vi "Main.vi"() -> ()   [LabVIEW 2021]
uses:
  Type defs/Parameters.ctl
  Type defs/Error FGV States.ctl
panel:
  out "image_num":i32
  in  "Stop":bool
  in  "Scanning options":enum32{"Item 0", "Item 1"}(radio)
  in  "Save to file":bool
  in  "Scanning":bool
  out "Errors":string
  in  "Saving data":T1
  out "Image Parameters":cluster{"Mean":dbl, "Offset":dbl}
  out "Intensity Graph":dbl[][](graph)
  in  "Parameters":T2={"Time"=0.0, "Pixels X"=1, "Pixels Y"=1, "Max galvo"=0.0, "Min galvo"=0.0} {"Pixels Y" min=1; "Pixels X" min=1 step=1; "Time" min=1.0}
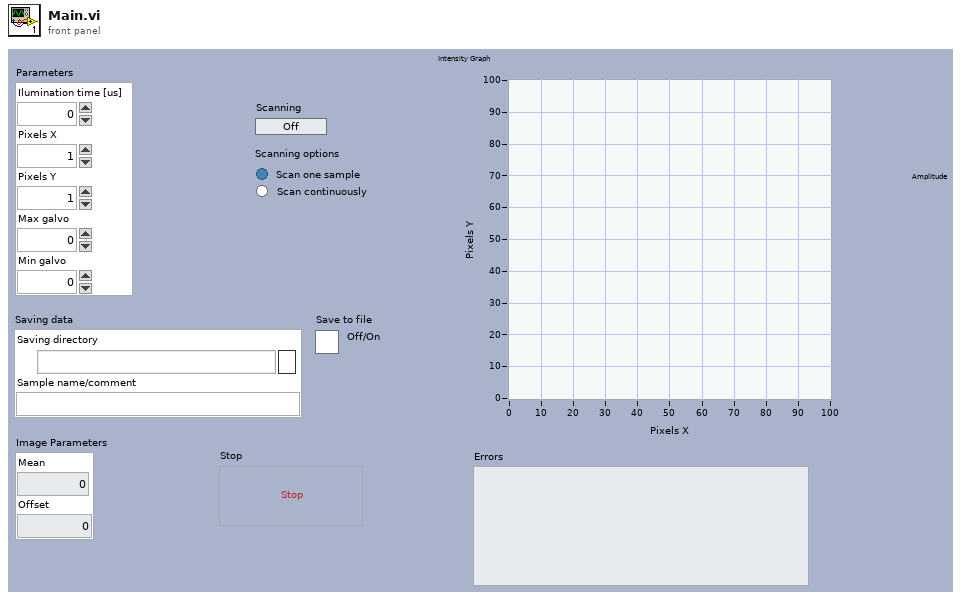
[diagram p1: front panel]
types:
  T1 = cluster{"Saving directory":path, "Sample name/comment":string}
  T2 = typedef "Parameters.ctl" = cluster{"Time":dbl, "Pixels X":i32, "Pixels Y":i32, "Max galvo":dbl, "Min galvo":dbl}
  T3 = typedef "Notifiers.ctl" = cluster{"DAQ notifier":refnum<notifier>, "Data notifier":refnum<notifier>}
  T4 = typedef "Queues.ctl" = cluster{"MHL":refnum<queue>, "DAQ":refnum<queue>, "Data":refnum<queue>, "Error":refnum<queue>}
  T5 = typedef "Error FGV States.ctl" = enum16{"Save", "Clear", "Add", "Read"}
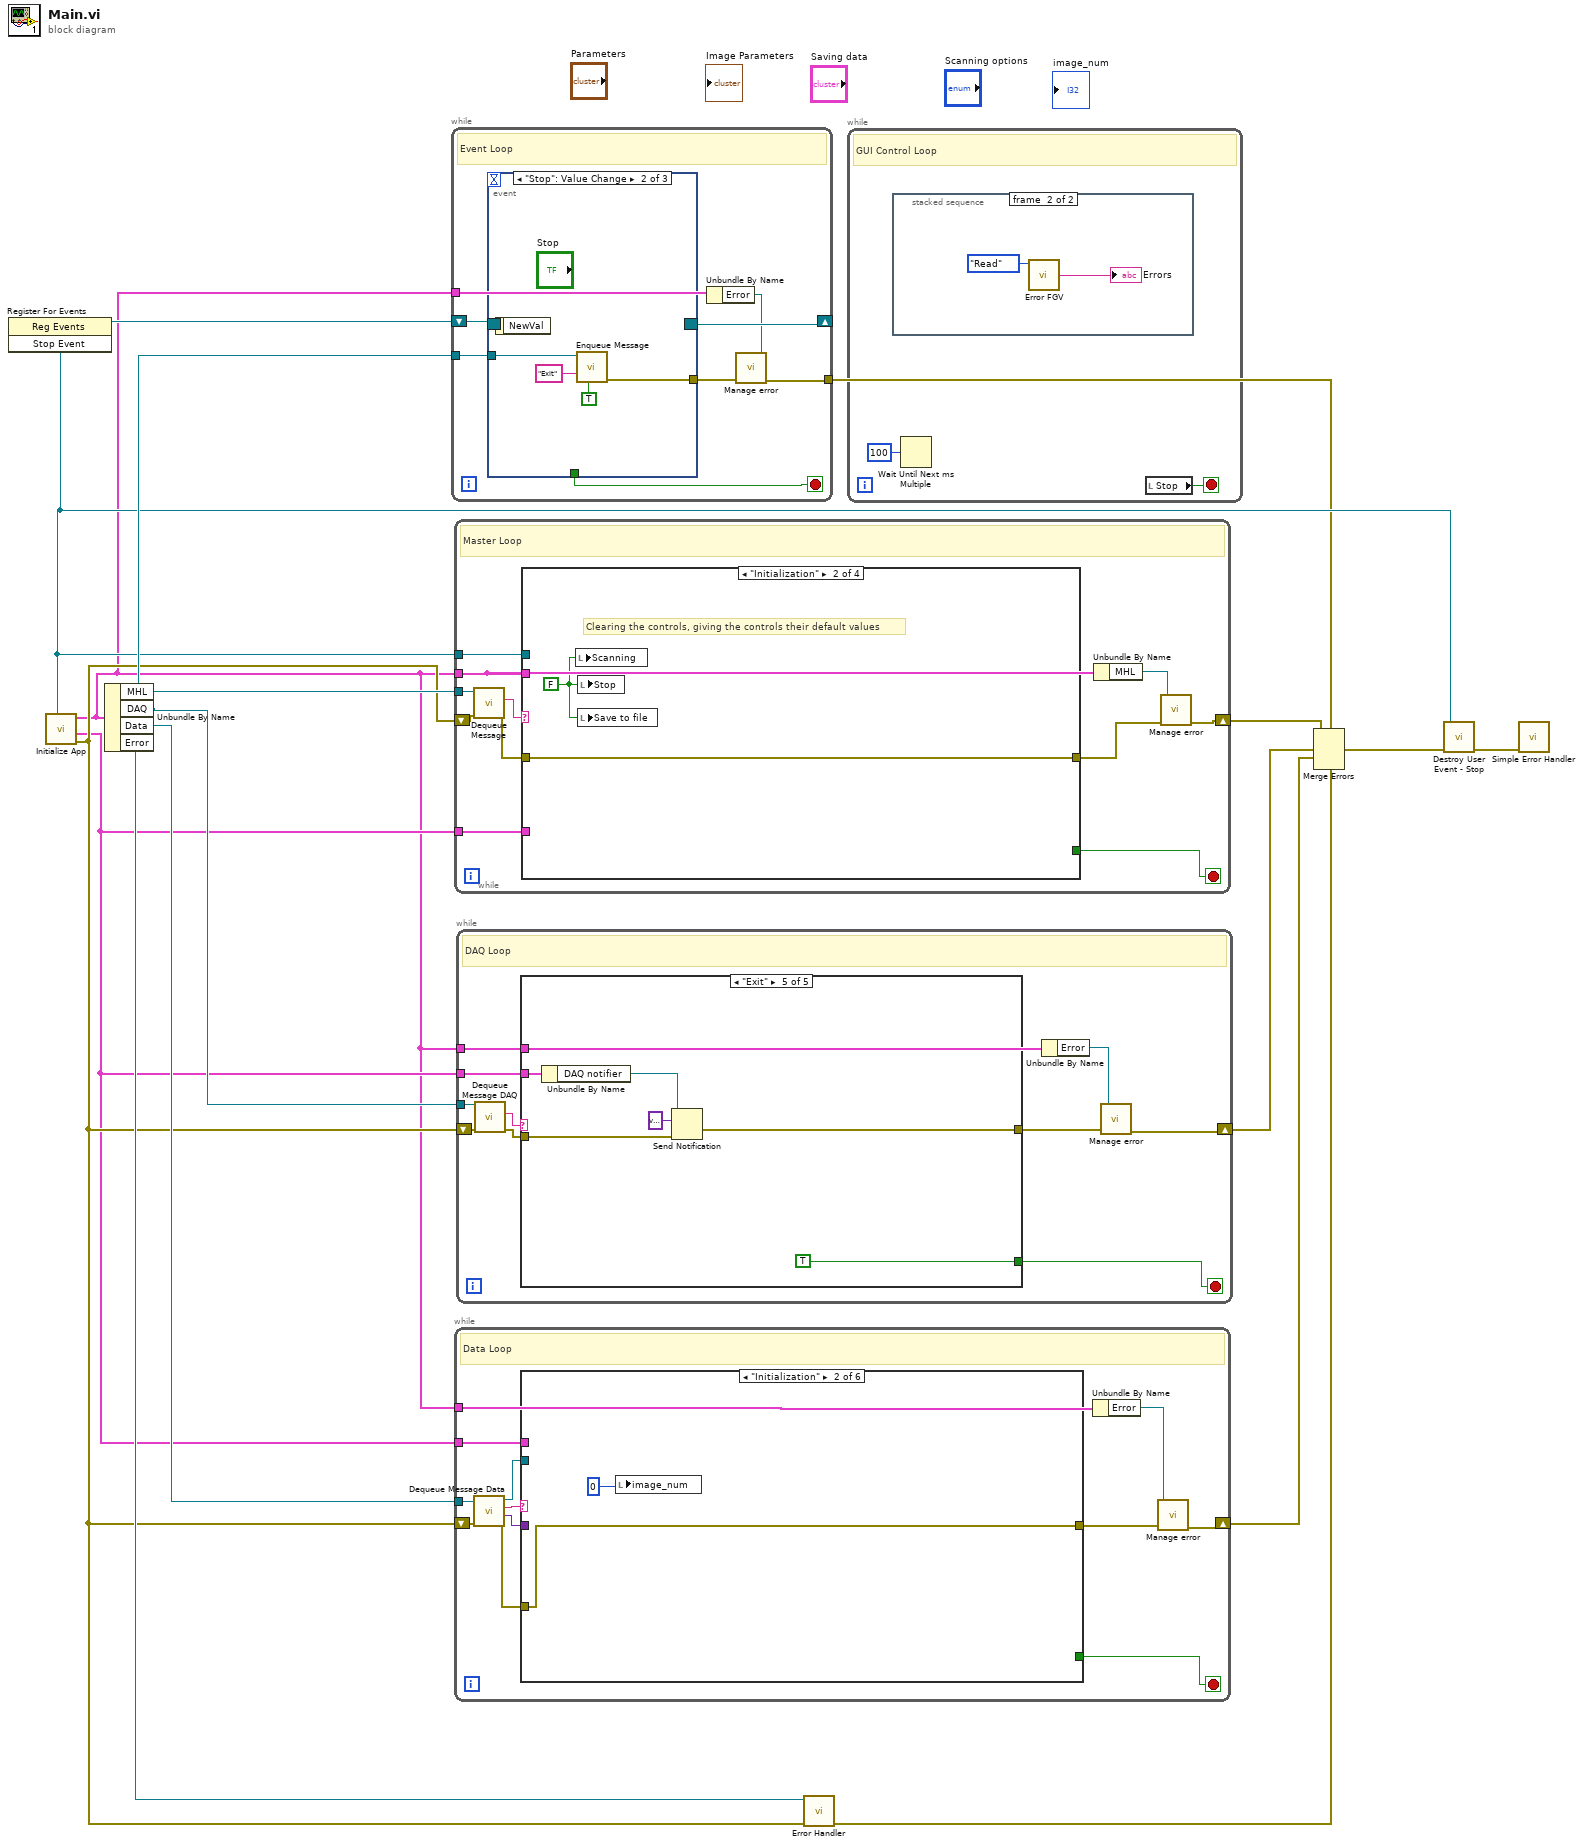
[diagram p0: block diagram]
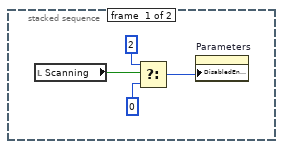
[diagram p2: hidden frame]
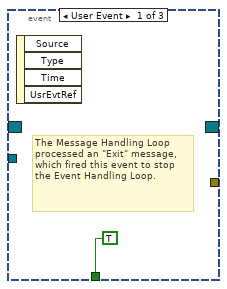
[diagram p3: hidden frame]
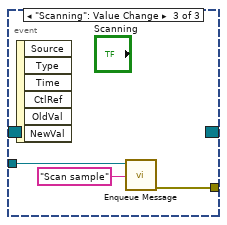
[diagram p4: hidden frame]
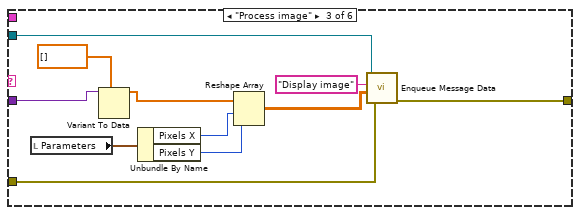
[diagram p6: hidden frame]
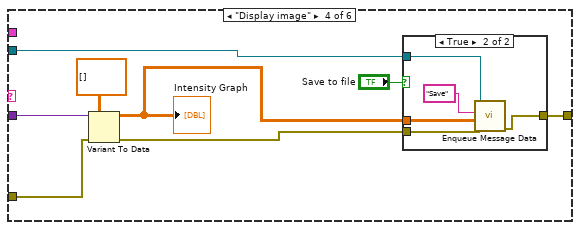
[diagram p7: hidden frame]
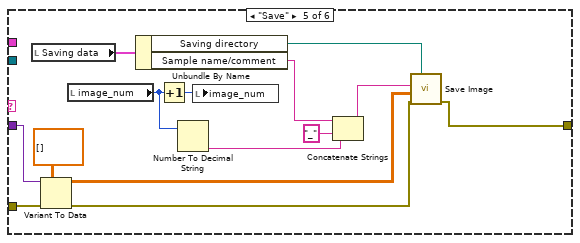
[diagram p9: hidden frame]
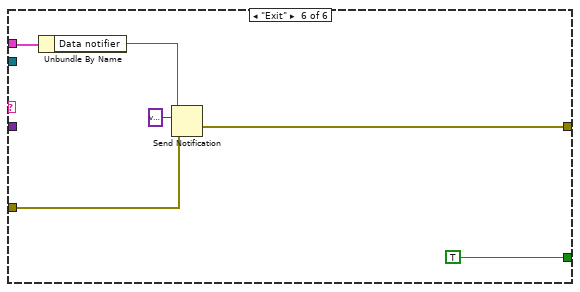
[diagram p10: hidden frame]
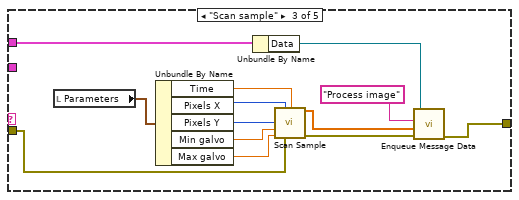
[diagram p13: hidden frame]
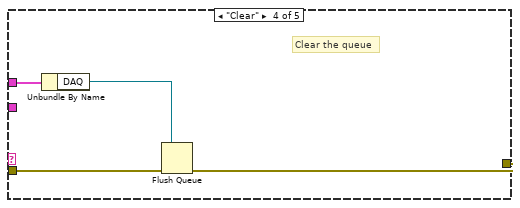
[diagram p14: hidden frame]
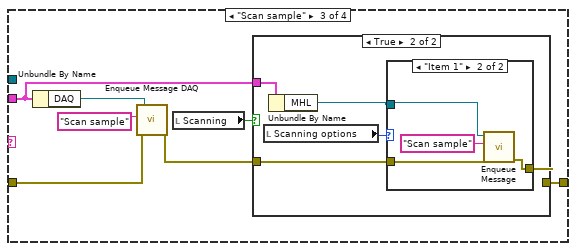
[diagram p16: hidden frame]
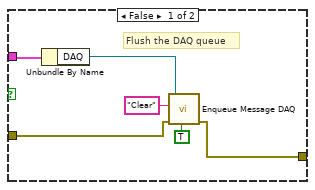
[diagram p17: hidden frame]
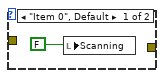
[diagram p18: hidden frame]
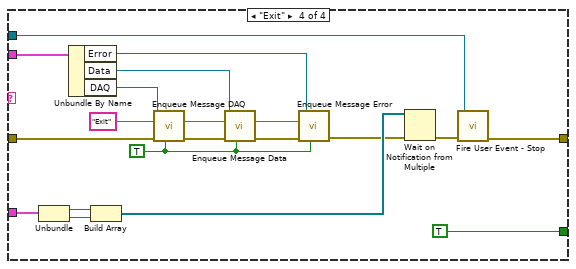
[diagram p19: hidden frame]
diagram:
  n1 = call "Initialize App.vi"() -> ("error out"=w10:errorcluster, "notifier cluster"=w2:T3, "Stop Event"=w11:refnum<user-event>, "queue cluster"=w1:T4)  [unwired: 8 in]
  n2 = register-events(w11) -> (reference out=w12:refnum<event-registration>)  [unwired: 2 in, 1 out]
  n3 = Unbundle By Name(w1) -> ("MHL"=w16:refnum<queue>, "DAQ"=w15:refnum<queue>, "Data"=w14:refnum<queue>, "Error"=w13:refnum<queue>)
  n4 = while {
    tunnel: w16 -> [w24]
    shift-right: [w22] -> _
    shift-left: w12 -> [w23]
    tunnel: [w19] -> w9
    tunnel: w1 -> [w18]
    stop <- w21 stop-if-true
    # "Event Loop"
    n5 = event shown="[1] \"Stop\": Value Change" {
      selector: w23 -> [_ _ _]
      dyn-events: [_ _ _] -> w22
      timeout: _ -> [_ _ _]
      tunnel: w24 -> [_ w29 w32]
      tunnel: [_ w28 w30] -> w20
      tunnel: [TRUE _ _] -> w21
      event User Event {
        # "The Message Handling Loop processed an \"Exit\" message, which fired this event to stop the Event Handling Loop."
        n6 = event-data() -> ()  [unwired: 1 in, 4 out]
      }
      event "Stop": Value Change {
        n7 = event-data() -> ()  [unwired: 1 in, 1 out]
        n8 = call "Enqueue Message.vi"("Priority message (F)"=TRUE, "Message"="Exit", "queue in"=w29) -> ("error out"=w28:errorcluster)  [unwired: 7 in, 1 out]
      }
      event "Scanning": Value Change {
        n9 = event-data() -> ()  [unwired: 1 in, 6 out]
        n10 = call "Enqueue Message.vi"("Message"="Scan sample", "queue in"=w32) -> ("error out"=w30:errorcluster)  [unwired: 8 in, 1 out]
      }
    }
    n11 = Unbundle By Name(w18) -> ("Error"=w17:refnum<queue>)
    n12 = call "Manage error.vi"("error in"=w20, "Error"=w17) -> ("error out"=w19:errorcluster)  [unwired: 9 in]
  }
  n13 = while {
    tunnel: w16 -> [w43]
    tunnel: w11 -> [w41]
    tunnel: w1 -> [w34]
    shift-right: [w35] -> w8
    shift-left: w10 -> [w38]
    tunnel: w2 -> [w37]
    stop <- w40 stop-if-true
    # "Master Loop"
    n14 = call "Dequeue Message.vi"("error in (no error)"=w38, "Message Queue"=w43) -> ("error out"=w39:errorcluster, "Message"=w42:string)  [unwired: 6 in, 2 out]
    n15 = case shown="\"Initialization\"" w42 {
      tunnel: w41 -> [_ _ _ w86]
      tunnel: [_ _ _ TRUE] -> w40
      tunnel: w34 -> [_ _ w49 w85]
      tunnel: w39 -> [w44 w46 w52 w79]
      tunnel: [w44 w46 w50 w76] -> w36
      tunnel: w37 -> [_ _ _ w75]
      frame Default {
      }
      frame "Initialization" {
        w45 = FALSE
        # "Clearing the controls, giving the controls their default values"
        n16 = local write "Scanning"(w45) -> ()
        n17 = local write "Stop"(w45) -> ()
        n18 = local write "Save to file"(w45) -> ()
      }
      frame "Scan sample" {
        n19 = Unbundle By Name(w49) -> ("DAQ"=w53:refnum<queue>)
        n20 = call "Enqueue Message DAQ.vi"("error in (no error)"=w52, "Message"="Scan sample", "queue in"=w53) -> ("error out"=w48:errorcluster)  [unwired: 7 in, 1 out]
        n21 = local read "Scanning"() -> (w47:bool)
        n22 = case shown="True" w47 {
          tunnel: [w56 w63] -> w50
          tunnel: w49 -> [w59 w62]
          tunnel: w48 -> [w57 w60]
          frame False {
            # "Flush the DAQ queue"
            n23 = Unbundle By Name(w59) -> ("DAQ"=w58:refnum<queue>)
            n24 = call "Enqueue Message DAQ.vi"("Priority message (F)"=TRUE, "error in (no error)"=w57, "Message"="Clear", "queue in"=w58) -> ("error out"=w56:errorcluster)  [unwired: 6 in, 1 out]
          }
          frame True {
            n25 = local read "Scanning options"() -> (w64:enum32{"Item 0", "Item 1"})
            n26 = Unbundle By Name(w62) -> ("MHL"=w61:refnum<queue>)
            n27 = case shown="\"Item 1\"" w64 {
              tunnel: [_ w69] -> w63
              tunnel: w61 -> [_ w68]
              tunnel: w60 -> [_ w66]
              frame "Item 0", Default {
                n28 = local write "Scanning"(FALSE) -> ()
              }
              frame "Item 1" {
                n29 = call "Enqueue Message.vi"("error in (no error)"=w66, "Message"="Scan sample", "queue in"=w68) -> ("error out"=w69:errorcluster)  [unwired: 7 in, 1 out]
              }
            }
          }
        }
      }
      frame "Exit" {
        w80 = TRUE ("Priority message (F)")
        w81 = "Exit"
        n30 = Unbundle(w75) -> ("DAQ notifier"=w74:refnum<notifier>, "Data notifier"=w73:refnum<notifier>)
        n31 = Unbundle By Name(w85) -> ("Error"=w82:refnum<queue>, "Data"=w83:refnum<queue>, "DAQ"=w84:refnum<queue>)
        n32 = Build Array(w74, w73) -> (w72:refnum<notifier>[])
        n33 = call "Enqueue Message DAQ.vi"("Priority message (F)"=w80, "error in (no error)"=w79, "Message"=w81, "queue in"=w84) -> ("error out"=w78:errorcluster)  [unwired: 6 in, 1 out]
        n34 = call "Enqueue Message Data.vi"("Priority message (F)"=w80, "error in (no error)"=w78, "Message"=w81, "queue in"=w83) -> ("error out"=w77:errorcluster)  [unwired: 6 in, 1 out]
        n35 = call "Enqueue Message Error.vi"("Priority message (F)"=w80, "error in (no error)"=w77, "Message"=w81, "queue in"=w82) -> ("error out"=w71:errorcluster)  [unwired: 6 in, 1 out]
        n36 = Wait on Notification from Multiple(0:w72, 3:w71) -> (11:w70:errorcluster)  [unwired: 2 in, 3 out]
        n37 = call "Fire User Event - Stop.vi"("error in (no error)"=w70, "Stop Event"=w86) -> ("error out"=w76:errorcluster)  [unwired: 9 in]
      }
    }
    n38 = Unbundle By Name(w34) -> ("MHL"=w33:refnum<queue>)
    n39 = call "Manage error.vi"("error in"=w36, "Error"=w33) -> ("error out"=w35:errorcluster)  [unwired: 9 in]
  }
  n40 = while {
    tunnel: w14 -> [w99]
    shift-right: [w90] -> w6
    shift-left: w10 -> [w96]
    tunnel: w2 -> [w92]
    tunnel: w1 -> [w89]
    stop <- w93 stop-if-true
    # "Data Loop"
    n41 = call "Dequeue Message Data.vi"("error in (no error)"=w96, "Message Queue"=w99) -> ("error out"=w94:errorcluster, "Data"=w97:variant, "Message"=w98:string, "dup Message Queue"=w95:refnum<queue>)  [unwired: 6 in]
    n42 = case shown="\"Initialization\"" w98 {
      tunnel: w97 -> [_ _ w110 w121 w135 _]
      tunnel: w95 -> [_ _ w107 w115 _ _]
      tunnel: w94 -> [w100 w102 w105 w119 w140 w144]
      tunnel: [w100 w102 w103 w116 w128 w143] -> w91
      tunnel: [_ _ _ _ _ TRUE] -> w93
      tunnel: w92 -> [_ _ _ _ _ w146]
      frame Default {
      }
      frame "Initialization" {
        n43 = local write "image_num"(0) -> ()
      }
      frame "Process image" {
        n44 = local read "Parameters"() -> (w113:T2)
        n45 = Variant To Data(type=dbl[] [] ("data"), Variant=w110) -> (data=w108:dbl[])  [unwired: 1 in, 1 out]
        n46 = Unbundle By Name(w113) -> ("Pixels X"=w112:i32, "Pixels Y"=w111:i32)
        n47 = Reshape Array(w108, w112, w111) -> (w104:dbl[][])
        n48 = call "Enqueue Message Data.vi"("error in (no error)"=w105, "Data"=w104, "Message"="Display image", "queue in"=w107) -> ("error out"=w103:errorcluster)  [unwired: 6 in, 1 out]
      }
      frame "Display image" {
        n49 = Variant To Data(error in=w119, type=dbl[][] [] ("output array"), Variant=w121) -> (data=w114:dbl[][], error out=w117:errorcluster)
        "Intensity Graph" <- w114
        n50 = case shown="True" "Save to file" {
          tunnel: w117 -> [w122 w127]
          tunnel: [w122 w126] -> w116
          tunnel: w115 -> [_ w125]
          tunnel: w114 -> [_ w124]
          frame False {
          }
          frame True {
            n51 = call "Enqueue Message Data.vi"("error in (no error)"=w127, "Data"=w124, "Message"="Save", "queue in"=w125) -> ("error out"=w126:errorcluster)  [unwired: 6 in, 1 out]
          }
        }
      }
      frame "Save" {
        n52 = local read "Saving data"() -> (w139:T1)
        n53 = Variant To Data(error in=w140, type=dbl[][] [] ("output array"), Variant=w135) -> (data=w137:dbl[][], error out=w136:errorcluster)
        n54 = local read "image_num"() -> (w133:i32)
        n55 = Unbundle By Name(w139) -> ("Saving directory"=w138:path, "Sample name/comment"=w132:string)
        n56 = Increment(x=w133) -> (x+1=w134:i32)
        n57 = Number To Decimal String(number=w133) -> (decimal integer string=w131:string)  [unwired: 1 in]
        n58 = local write "image_num"(w134) -> ()
        n59 = Concatenate Strings(w132, "_" ("string"), w131) -> (w129:string)
        n60 = call "Save Image.vi"("error in"=w136, "Measurements"=w137, "Sample name"=w129, "base path"=w138) -> ("error out"=w128:errorcluster)  [unwired: 7 in]
      }
      frame "Exit" {
        n61 = Unbundle By Name(w146) -> ("Data notifier"=w145:refnum<notifier>)
        n62 = Send Notification(notification=variant, notifier=w145, error in (no error)=w144) -> (error out=w143:errorcluster)  [unwired: 1 out]
      }
    }
    n63 = Unbundle By Name(w89) -> ("Error"=w88:refnum<queue>)
    n64 = call "Manage error.vi"("error in"=w91, "Error"=w88) -> ("error out"=w90:errorcluster)  [unwired: 9 in]
  }
  n65 = while {
    tunnel: w15 -> [w157]
    tunnel: w1 -> [w148]
    shift-right: [w150] -> w7
    shift-left: w10 -> [w155]
    tunnel: w2 -> [w152]
    stop <- w154 stop-if-true
    # "DAQ Loop"
    n66 = call "Dequeue Message DAQ.vi"("error in (no error)"=w155, "Message Queue"=w157) -> ("error out"=w153:errorcluster, "Message"=w156:string)  [unwired: 6 in, 2 out]
    n67 = case shown="\"Exit\"" w156 {
      tunnel: w148 -> [_ _ w166 w176 _]
      tunnel: [_ _ _ _ TRUE] -> w154
      tunnel: w153 -> [w158 w159 w161 w173 w181]
      tunnel: [w158 w159 w160 w174 w180] -> w151
      tunnel: w152 -> [_ _ _ _ w179]
      frame Default {
      }
      frame "Initialization" {
      }
      frame "Scan sample" {
        n68 = local read "Parameters"() -> (w172:T2)
        n69 = Unbundle By Name(w172) -> ("Time"=w171:dbl, "Pixels X"=w170:i32, "Pixels Y"=w169:i32, "Min galvo"=w168:dbl, "Max galvo"=w167:dbl)
        n70 = Unbundle By Name(w166) -> ("Data"=w165:refnum<queue>)
        n71 = call "Scan Sample.vi"("Czas naœwietlania (us)"=w171, "pixels x"=w170, "pixels y"=w169, "Zakres skanowania min"=w168, "Zakres skanowania max"=w167, "error in"=w161) -> ("data"=w164:dbl[], "error out"=w163:errorcluster)  [unwired: 8 in]
        n72 = call "Enqueue Message Data.vi"("error in (no error)"=w163, "Data"=w164, "Message"="Process image", "queue in"=w165) -> ("error out"=w160:errorcluster)  [unwired: 6 in, 1 out]
      }
      frame "Clear" {
        # "Clear the queue"
        n73 = Unbundle By Name(w176) -> ("DAQ"=w175:refnum<queue>)
        n74 = Flush Queue(queue=w175, error in (no error)=w173) -> (error out=w174:errorcluster)  [unwired: 2 out]
      }
      frame "Exit" {
        n75 = Unbundle By Name(w179) -> ("DAQ notifier"=w178:refnum<notifier>)
        n76 = Send Notification(notification=variant, notifier=w178, error in (no error)=w181) -> (error out=w180:errorcluster)  [unwired: 1 out]
      }
    }
    n77 = Unbundle By Name(w148) -> ("Error"=w149:refnum<queue>)
    n78 = call "Manage error.vi"("error in"=w151, "Error"=w149) -> ("error out"=w150:errorcluster)  [unwired: 9 in]
  }
  n79 = call "Error Handler.vi"("error in (no error)"=w10, "queue"=w13) -> ("error out"=w5:errorcluster)  [unwired: 8 in, 1 out]
  n80 = while {
    stop <- w183 stop-if-true
    # "GUI Control Loop"
    n81 = stacked-sequence {
      frame #0 {
        n82 = local read "Scanning"() -> (w185:bool)
        n83 = Select(t=2, s=w185, f=0) -> (s? t:f=w188:i32)
        n84 = property on="Parameters" class="Clust (strict)"("DisabledEnum"=w188) -> ()  [unwired: 2 in, 2 out]
      }
      frame #1 {
        n85 = call "Error FGV.vi"("FGV states"=Error_FGV_States."Read") -> ("Errors"=→"Errors":string)  [unwired: 10 in]
      }
    }
    n86 = Wait Until Next ms Multiple(millisecond multiple=u32 100) -> ()  [unwired: 1 out]
    n87 = local read "Stop"() -> (w183:bool)
  }
  n88 = Merge Errors(w9, w8, w7, w6, w5) -> (w3:errorcluster)
  n89 = call "Destroy User Event - Stop.vi"("error in (no error)"=w3, "Stop Event"=w11) -> ("error out"=w4:errorcluster)  [unwired: 9 in]
  n90 = call <vilib>:"Simple Error Handler.vi"("error in (no error)"=w4) -> ()  [unwired: 4 in, 5 out]
